vi "OverlayArcCenterSize.vi"(4 "Color":u32(colorbox)=16711680, 5 "GroupName":string, 6 "Drawing Mode (Fill)":T3=enum."Fill", 7 "Angles":T1 {"End Angle (degrees)" format="%.2f"; "Start Angle (degrees)" format="%.2f"}, 8 "error in":errorcluster, 9 "Size":T2, 10 "Center-Point":T2, 11 "Image Reference In":T4) -> (0 "error out":errorcluster, 3 "Image Reference Out":T4)   [LabVIEW 2020, in "OpenLvVision_Overlays.lvlib"]
doc: "Overlay a arc on top of an image.\nDraws the arc arround a center point."
uses:
  OpenLvVision_Overlays.lvlib
  <vilib>/OpenLvVision/OpenLvVision_Image/Management/TypeDef/OLV Image.ctl
  <vilib>/OpenLvVision/OpenLvVision_Image/Management/OLV Management.lvlib
  TypeDefs/DrawingMode.ctl
  TypeDefs/PointI32.ctl
  TypeDefs/Angles.ctl
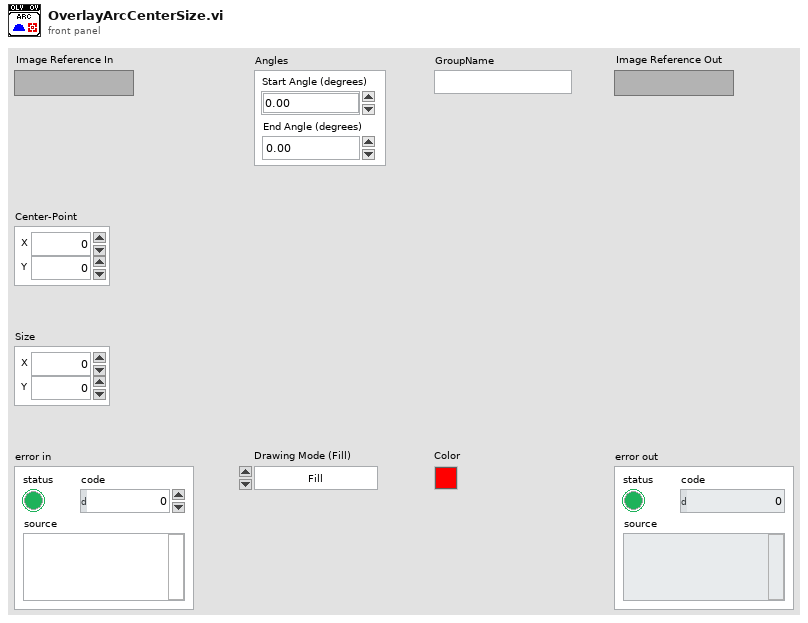
[diagram p1: front panel]
types:
  T1 = typedef "OpenLvVision_Overlays.lvlib/Angles.ctl" = cluster{"Start Angle (degrees)":dbl, "End Angle (degrees)":dbl}
  T2 = typedef "OpenLvVision_Overlays.lvlib/PointI32.ctl" = cluster{"X":i32, "Y":i32}
  T3 = typedef "OpenLvVision_Overlays.lvlib/DrawingMode.ctl" = enum16{"Frame", "Fill"}
  T4 = typedef "OLV OpenLvVision_Image.lvlib/OLV Management.lvlib/OLV Image.ctl" = refnum<image>
  T5 = typedef "OLV OpenLvVision_Image.lvlib/OLV DataAccess.lvlib/OLV RectangleI32.ctl" = cluster{"Left":i32, "Top":i32, "Right":i32, "Bottom":i32}
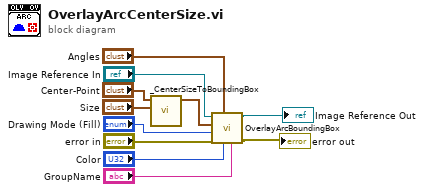
[diagram p0: block diagram]
diagram:
  n1 = call "_CenterSizeToBoundingBox.vi"("Size"="Size", "Center-Point"="Center-Point") -> ("Bounding Box"=w2:T5)  [unwired: 9 in]
  n2 = call "OverlayArcBoundingBox.vi"("GroupName"="GroupName", "Color"="Color", "Angles"="Angles", "error in"="error in", "Drawing Mode (Frame)"="Drawing Mode (Fill)", "BondingBox"=w2, "Image Reference In"="Image Reference In") -> ("error out"=→"error out":errorcluster, "Image Reference Out"=→"Image Reference Out":T4)  [unwired: 3 in]
